vi "_Highlight CSM Scripts(StringControl).vi"(11 "String Ctrl":refnum<vi>) -> (3 "String Ctrl (Dup)":refnum<vi>)   [LabVIEW 2017]
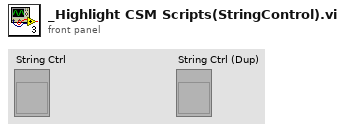
[diagram p1: front panel]
types:
  T1 = cluster{"Text.Selection:Start":u32, "Text.Selection:End":u32, "cb":u32, "underline":bool, "Italic":bool, "Bold":bool}[]
  T2 = typedef "LVSelectionTypeDef.ctl" = cluster{"Selection Start":u32, "Selection End":u32}
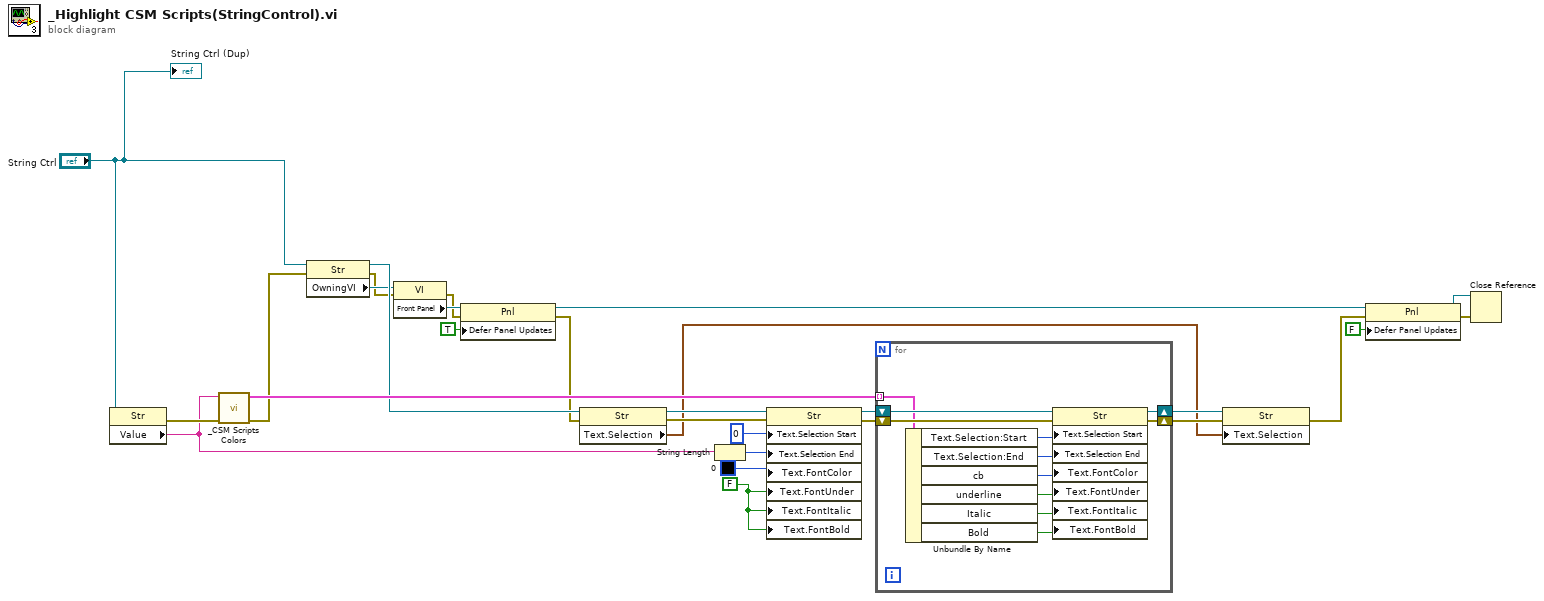
[diagram p0: block diagram]
diagram:
  w20 = FALSE ("Text.Font:Underline")
  n1 = property class="Str"(reference="String Ctrl") -> (error out=w28:errorcluster, "Value"=w22:string)  [unwired: 1 in, 1 out]
  n2 = call "_CSM Scripts Colors.vi"("Error In"=w28, "Value"=w22) -> ("error out"=w16:errorcluster, "Array"=w27:T1)  [unwired: 8 in]
  n3 = property class="Str"(reference="String Ctrl", error in=w16) -> (reference out=w19:refnum<vi>, error out=w13:errorcluster, "OwningVI"=w18:refnum<vi>)
  n4 = property class="VI"(reference=w18, error in=w13) -> (error out=w14:errorcluster, "Front Panel"=w17:refnum<vi>)  [unwired: 1 out]
  n5 = property class="Pnl"(reference=w17, error in=w14, "Defer Panel Updates"=TRUE) -> (reference out=w11:refnum<vi>, error out=w6:errorcluster)
  n6 = property class="Str"(reference=w19, error in=w6) -> (reference out=w7:refnum<vi>, error out=w5:errorcluster, "Text.Selection"=w1:T2)
  n7 = String Length(string=w22) -> (length=w23:i32)
  n8 = property class="Str"(reference=w7, error in=w5, "Text.Selection Start"=u32 0 ("Text.Selection:Start"), "Text.Selection End"=w23, "Text.FontColor"=u32 0, "Text.FontUnder"=w20, "Text.FontItalic"=w20, "Text.FontBold"=w20) -> (reference out=w25:refnum<vi>, error out=w26:errorcluster)
  n9 = for {
    tunnel: w27 -> [w37] mode=indexing
    shift-right: [w30] -> w4
    shift-left: w26 -> [w38]
    shift-right: [w29] -> w2
    shift-left: w25 -> [w39]
    n10 = Unbundle By Name(w37) -> ("Text.Selection:Start"=w36:u32, "Text.Selection:End"=w35:u32, "cb"=w34:u32, "underline"=w33:bool, "Italic"=w32:bool, "Bold"=w31:bool)
    n11 = property class="Str"(reference=w39, error in=w38, "Text.Selection Start"=w36, "Text.Selection End"=w35, "Text.FontColor"=w34, "Text.FontUnder"=w33, "Text.FontItalic"=w32, "Text.FontBold"=w31) -> (reference out=w29:refnum<vi>, error out=w30:errorcluster)
  }
  n12 = property class="Str"(reference=w2, error in=w4, "Text.Selection"=w1) -> (error out=w3:errorcluster)  [unwired: 1 out]
  n13 = property class="Pnl"(reference=w11, error in=w3, "Defer Panel Updates"=FALSE) -> (reference out=w9:refnum<vi>, error out=w10:errorcluster)
  n14 = Close Reference(reference=w9, error in (no error)=w10) -> ()  [unwired: 1 out]
  "String Ctrl (Dup)" <- "String Ctrl"
